vi "XPN Acquire Software Defect Frames.vi"(8 "error in (no error)":errorcluster, 11 "numFrames":i32) -> (0 "error out":errorcluster, 3 "function return":i32)   [LabVIEW 2025, in "xPanelWrapper.lvlib"]
doc: "XPN_API int XPN_AcquireSoftwareDefectFrames(int numFrames);"
uses:
  xPanelWrapper.lvlib
  xPanelWrapper.dll
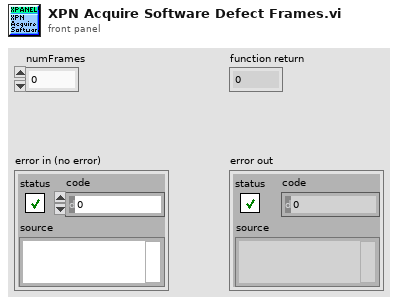
[diagram p1: front panel]
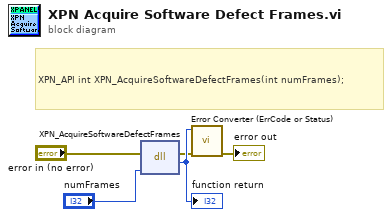
[diagram p0: block diagram]
diagram:
  # "XPN_API int XPN_AcquireSoftwareDefectFrames(int numFrames);"
  n1 = dll-call lib="E:/GitHub/xPanelWrapper/xPanelWrapperLvLib/xPanelWrapper.*" fn="XPN_AcquireSoftwareDefectFrames"(error in="error in (no error)", "numFrames"="numFrames") -> (error out=w2:errorcluster, w5:i32)  [unwired: 3 in, 1 out]
  "function return" <- w5
  n2 = call "Error Converter (ErrCode or Status).vi"("error in (no error)"=w2, "error code"=w5) -> ("error out"=→"error out":errorcluster)  [unwired: 9 in]
